vi "Format EoL for CSV.vi"(9 "Is System Encoding (f)":bool, 11 "String In":string) -> (3 "String":string)   [LabVIEW 2019, in "Language Editor.lvlib"]
doc: "- - -\nCopyright (c) 2026, Merecs Engineering GmbH"
uses:
  Language Editor.lvlib
panel:
  # "Connector Pane"
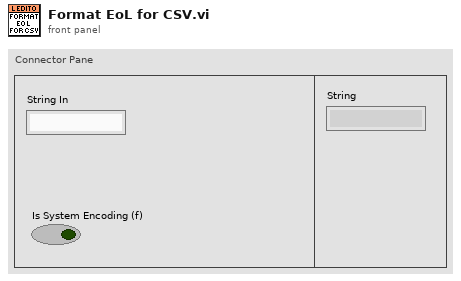
[diagram p1: front panel]
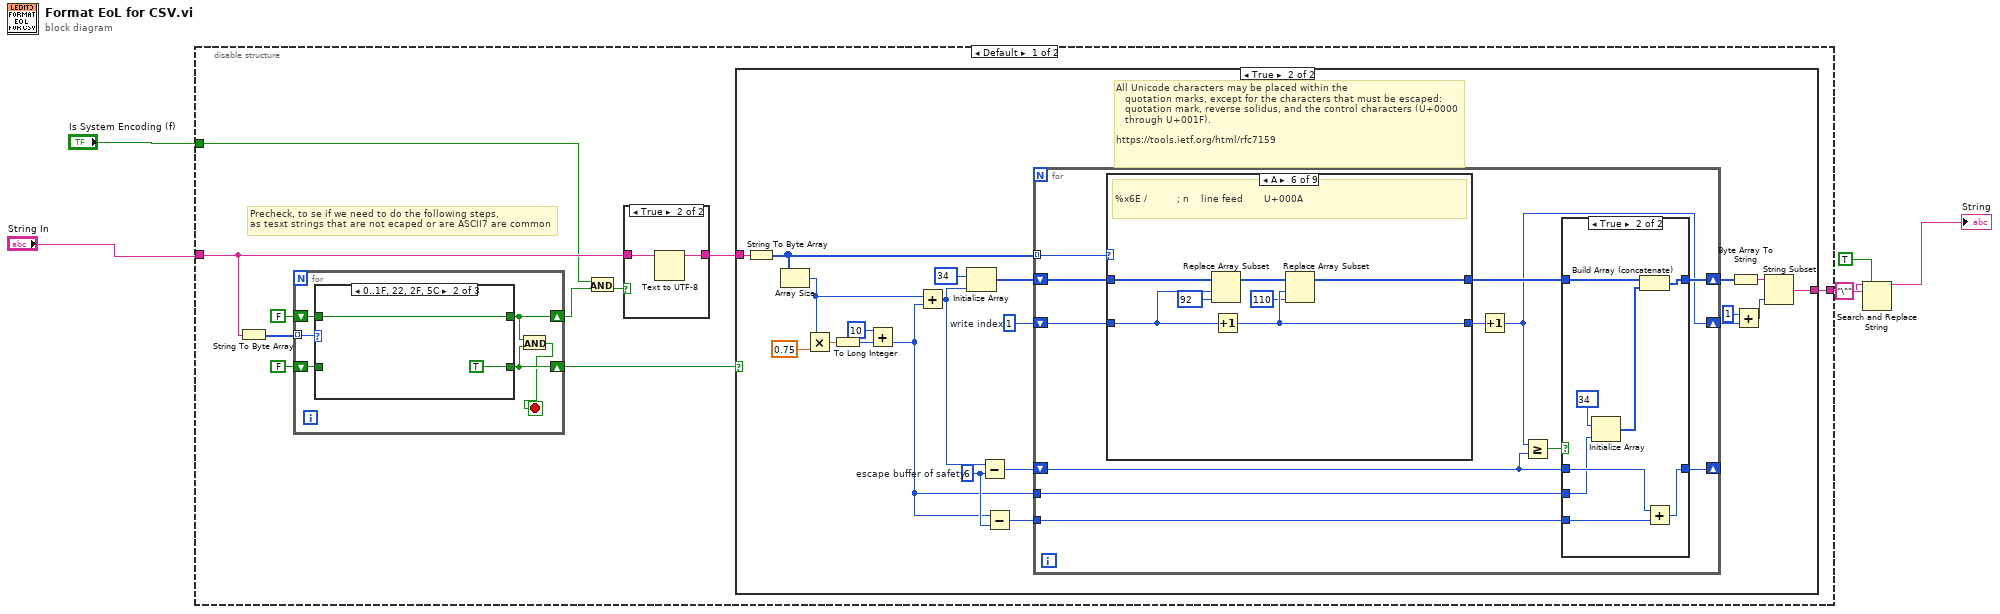
[diagram p0: block diagram]
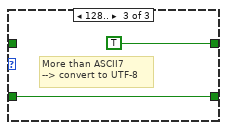
[diagram p4: hidden frame]
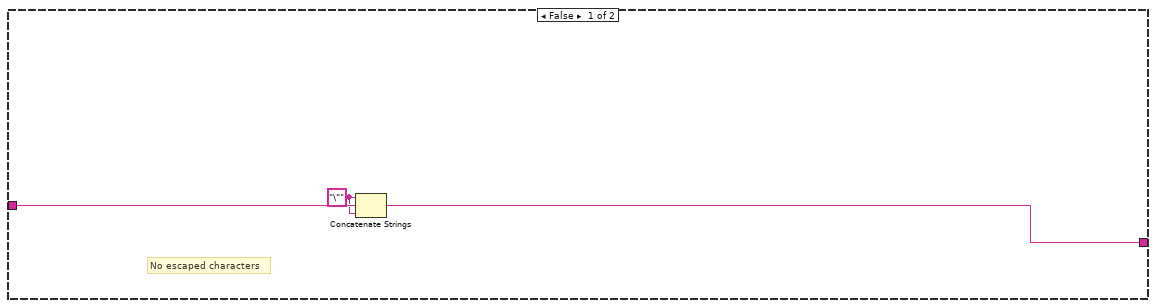
[diagram p5: hidden frame]
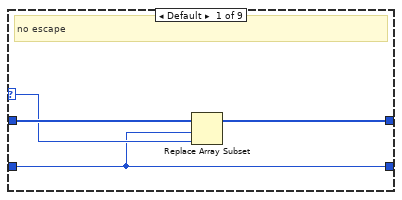
[diagram p7: hidden frame]
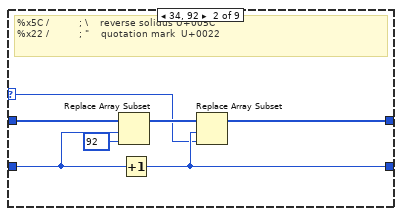
[diagram p8: hidden frame]
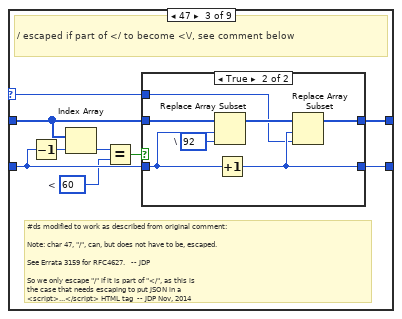
[diagram p9: hidden frame]
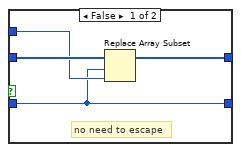
[diagram p10: hidden frame]
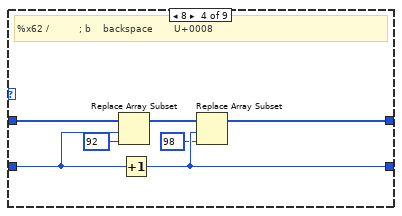
[diagram p11: hidden frame]
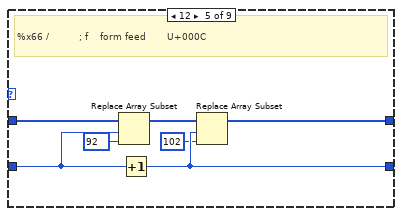
[diagram p12: hidden frame]
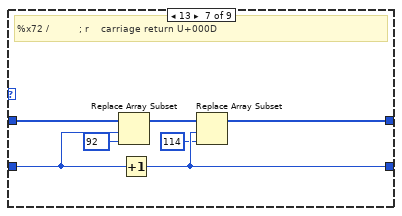
[diagram p13: hidden frame]
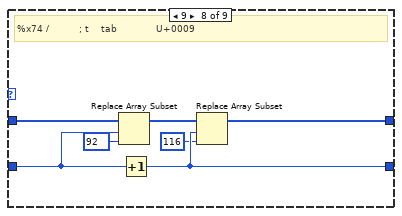
[diagram p14: hidden frame]
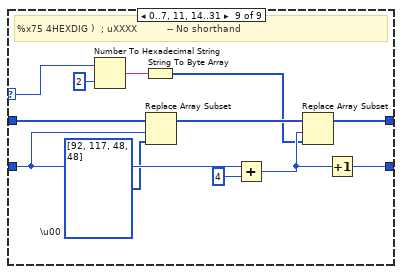
[diagram p15: hidden frame]
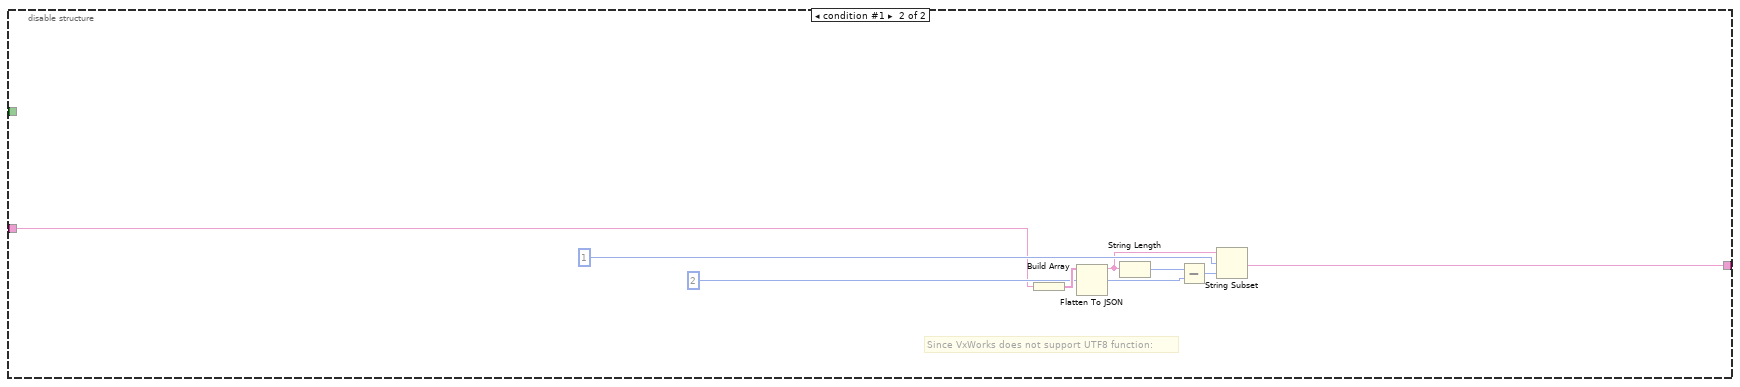
[diagram p16: hidden frame]
diagram:
  n1 = disable-structure shown="Default" {
    disable-tunnel: [w16 w157] -> w3
    disable-tunnel: "String In" -> [w14 w156]
    disable-tunnel: "Is System Encoding (f)" -> [w7 _]
    frame condition #0 (active) {
      # "Precheck, to se if we need to do the following steps,\nas tesxt strings that are not ecaped or are ASCII7 are common"
      n2 = String To Byte Array(string=w14) -> (unsigned byte array=w12:u8[])
      n3 = for {
        tunnel: w12 -> [w25] mode=indexing
        shift-right: [w24] -> w9
        shift-left: FALSE -> [w21]
        shift-right: [w23] -> w13
        shift-left: FALSE -> [w20]
        stop <- w22 stop-if-true
        n4 = case shown="0..1F, 22, 2F, 5C" w25 {
          tunnel: [w27 w28 TRUE] -> w24
          tunnel: [w26 TRUE w30] -> w23
          tunnel: w21 -> [w27 w28 _]
          tunnel: w20 -> [w26 _ w30]
          frame Default {
          }
          frame 0..31, 34, 47, 92 {
          }
          frame 128.. {
            # "More than ASCII7\n--> convert to UTF-8"
          }
        }
        n5 = And(x=w24, y=w23) -> (x .and. y?=w22:bool)
      }
      n6 = And(x=w7, y=w9) -> (x .and. y?=w8:bool)
      n7 = case shown="True" w8 {
        tunnel: [w17 w19] -> w15
        tunnel: w14 -> [w17 w18]
        frame False {
        }
        frame True {
          n8 = Text to UTF-8(11:w18) -> (3:w19:string)  [unwired: 2 in, 1 out]
        }
      }
      n9 = case shown="True" w13 {
        tunnel: [w33 w55] -> w16
        tunnel: w15 -> [w34 w35]
        frame False {
          w32 = "\"" ("string")
          # "No escaped characters"
          n10 = Concatenate Strings(w32, w34, w32) -> (w33:string)
        }
        frame True {
          w41 = 6  # escape buffer of safety
          w53 = 1  # write index
          # "All Unicode characters may be placed within the\n   quotation marks, except for the characters that must be escaped:\n   quotation mark, reverse solidus, and the control characters (U+0000\n   through U+001F).\n\nhttps://tools.ietf.org/html/rfc7159"
          n11 = String To Byte Array(string=w35) -> (unsigned byte array=w47:u8[])
          n12 = Array Size(array=w47) -> (size(s)=w45:i32)
          n13 = Multiply(x=w45, y=0.75) -> (x*y=w48:dbl)
          n14 = To Long Integer(number=w48) -> (32bit integer=w42:i32)
          n15 = Add(x=10, y=w42) -> (x+y=w38:i32)
          n16 = Add(x=w45, y=w38) -> (x+y=w44:i32)
          n17 = Initialize Array(u8 34, w44) -> (w50:u8[])
          n18 = Subtract(x=w44, y=w41) -> (x-y=w43:i32)
          n19 = Subtract(x=w38, y=w41) -> (x-y=w40:i32)
          n20 = for {
            shift-right: [w64] -> w52
            shift-left: w50 -> [w67]
            shift-right: [w57] -> w46
            shift-left: w53 -> [w66]
            tunnel: w47 -> [w65] mode=indexing
            shift-right: [w61] -> _
            shift-left: w43 -> [w60]
            tunnel: w38 -> [w59]
            tunnel: w40 -> [w58]
            n21 = case shown="A" w65 {
              selector: w65 -> [w79 w83 w95 _ _ _ _ _ w152]
              tunnel: w67 -> [w81 w88 w94 w115 w122 w129 w136 w143 w155]
              tunnel: [w80 w85 w97 w112 w119 w126 w133 w140 w154] -> w63
              tunnel: w66 -> [w78 w86 w93 w113 w120 w127 w134 w141 w153]
              tunnel: [w78 w84 w96 w111 w118 w125 w132 w139 w144] -> w62
              frame Default {
                # "no escape"
                n22 = Replace Array Subset(array=w81, new element=w79, index=w78) -> (w80:u8[])
              }
              frame 34, 92 {
                # "%x5C /          ; \\    reverse solidus U+005C\n%x22 /          ; \"    quotation mark  U+0022"
                n23 = Replace Array Subset(array=w88, new element=u8 92 ("new element/subarray"), index=w86) -> (w87:u8[])
                n24 = Increment(x=w86) -> (x+1=w84:i32)
                n25 = Replace Array Subset(array=w87, new element=w83, index=w84) -> (w85:u8[])
              }
              frame 47 {
                w89 = u8 60  # <
                # "#ds modified to work as described from original comment:\n\nNote: char 47, \"/\", can, but does not have to be, escaped.\n\nSee Errata 3159 for RFC4627.   -- JDP\n\nSo we only escape \"/\" if it is part of \"</\", as this is\nthe case that needs escaping to put JSON in a\n<script>...</script> HTML tag  -- JDP Nov, 2014"
                # "/ escaped if part of </ to become <\\/, see comment below"
                n26 = Decrement(x=w93) -> (x-1=w92:i32)
                n27 = Index Array(array=w94, index=w92) -> (element=w91:u8)
                n28 = Equal?(x=w91, y=w89) -> (x = y?=w90:bool)
                n29 = case shown="True" w90 {
                  tunnel: [w100 w107] -> w97
                  tunnel: [w98 w106] -> w96
                  tunnel: w95 -> [w99 w105]
                  tunnel: w94 -> [w101 w104]
                  tunnel: w93 -> [w98 w103]
                  frame False {
                    # "no need to escape"
                    n30 = Replace Array Subset(array=w101, new element=w99, index=w98) -> (w100:u8[])
                  }
                  frame True {
                    w102 = u8 92  # \
                    n31 = Replace Array Subset(array=w104, new element=w102, index=w103) -> (w108:u8[])
                    n32 = Increment(x=w103) -> (x+1=w106:i32)
                    n33 = Replace Array Subset(array=w108, new element=w105, index=w106) -> (w107:u8[])
                  }
                }
              }
              frame 8 {
                # "%x62 /          ; b    backspace       U+0008"
                n34 = Replace Array Subset(array=w115, new element=u8 92 ("new element/subarray"), index=w113) -> (w114:u8[])
                n35 = Increment(x=w113) -> (x+1=w111:i32)
                n36 = Replace Array Subset(array=w114, new element=u8 98 ("new element/subarray"), index=w111) -> (w112:u8[])
              }
              frame 12 {
                # "%x66 /          ; f    form feed       U+000C"
                n37 = Replace Array Subset(array=w122, new element=u8 92 ("new element/subarray"), index=w120) -> (w121:u8[])
                n38 = Increment(x=w120) -> (x+1=w118:i32)
                n39 = Replace Array Subset(array=w121, new element=u8 102 ("new element/subarray"), index=w118) -> (w119:u8[])
              }
              frame 10 {
                # "%x6E /          ; n    line feed       U+000A"
                n40 = Replace Array Subset(array=w129, new element=u8 92 ("new element/subarray"), index=w127) -> (w128:u8[])
                n41 = Increment(x=w127) -> (x+1=w125:i32)
                n42 = Replace Array Subset(array=w128, new element=u8 110 ("new element/subarray"), index=w125) -> (w126:u8[])
              }
              frame 13 {
                # "%x72 /          ; r    carriage return U+000D"
                n43 = Replace Array Subset(array=w136, new element=u8 92 ("new element/subarray"), index=w134) -> (w135:u8[])
                n44 = Increment(x=w134) -> (x+1=w132:i32)
                n45 = Replace Array Subset(array=w135, new element=u8 114 ("new element/subarray"), index=w132) -> (w133:u8[])
              }
              frame 9 {
                # "%x74 /          ; t    tab             U+0009"
                n46 = Replace Array Subset(array=w143, new element=u8 92 ("new element/subarray"), index=w141) -> (w142:u8[])
                n47 = Increment(x=w141) -> (x+1=w139:i32)
                n48 = Replace Array Subset(array=w142, new element=u8 116 ("new element/subarray"), index=w139) -> (w140:u8[])
              }
              frame 0..7, 11, 14..31 {
                w145 = u8[] [92, 117, 48, 48]  # \u00
                # "%x75 4HEXDIG )  ; uXXXX          -- No shorthand"
                n49 = Number To Hexadecimal String(1:i16 2 ("width (-)"), 2:w152) -> (0:w147:string)
                n50 = String To Byte Array(string=w147) -> (unsigned byte array=w149:u8[])
                n51 = Replace Array Subset(array=w155, new element=w145, index=w153) -> (w151:u8[])
                n52 = Add(x=w153, y=4) -> (x+y=w150:i32)
                n53 = Replace Array Subset(array=w151, new element=w149, index=w150) -> (w154:u8[])
                n54 = Increment(x=w150) -> (x+1=w144:i32)
              }
            }
            n55 = Increment(x=w62) -> (x+1=w57:i32)
            n56 = Greater Or Equal?(x=w57, y=w60) -> (x >= y?=w56:bool)
            n57 = case shown="True" w56 {
              tunnel: [w69 w72] -> w64
              tunnel: w63 -> [w69 w73]
              tunnel: [w68 w75] -> w61
              tunnel: w60 -> [w68 w76]
              tunnel: w59 -> [_ w74]
              tunnel: w58 -> [_ w77]
              frame False {
              }
              frame True {
                n58 = Initialize Array(u8 34, w74) -> (w71:u8[])
                n59 = Build Array (concatenate)(w73, w71) -> (w72:u8[])
                n60 = Add(x=w76, y=w77) -> (x+y=w75:i32)
              }
            }
          }
          n61 = Byte Array To String(unsigned byte array=w52) -> (string=w54:string)
          n62 = Add(x=1, y=w46) -> (x+y=w39:i32)
          n63 = String Subset(string=w54, length (rest)=w39) -> (substring=w55:string)  [unwired: 1 in]
        }
      }
    }
    frame condition #1 {
      # "Since VxWorks does not support UTF8 function:"
      n64 = Build Array(w156) -> (w163:string[])
      n65 = Flatten To JSON(anything=w163) -> (JSON string=w160:string)  [unwired: 2 in, 1 out]
      n66 = String Length(string=w160) -> (length=w161:i32)
      n67 = Subtract(x=w161, y=2 ("x")) -> (x-y=w159:i32)
      n68 = String Subset(string=w160, offset (0)=1, length (rest)=w159) -> (substring=w157:string)
    }
  }
  n69 = Search and Replace String(replace all?=TRUE ("replace all? (F)"), input string=w3, search string="\"") -> (result string=→"String":string)  [unwired: 5 in, 3 out]
